vi "Test MQTT-3.1.2-1.vi"(8 "error in (no error)":errorcluster, 11 "Connection Config":refnum<class "Connection.lvclass">) -> (0 "error out":errorcluster, 3 "Connection Config dup":refnum<class "Connection.lvclass">)   [LabVIEW 2013]
uses:
  <vilib>/LabVIEW Open Source Project/MQTT Control Packets/Control Packets/CONNECT/CONNECT.lvclass
  <vilib>/LabVIEW Open Source Project/MQTT Control Packets/Control Packets/ControlPacket/ControlPacket.lvclass
  <vilib>/addons/_JKI Toolkits/Caraya/classes/Test/Test.lvclass
  <vilib>/addons/_JKI Toolkits/Caraya/classes/Assert/Assert.lvclass
  <vilib>/LabVIEW Open Source Project/Connection/Connection/Connection.lvclass
  <vilib>/LabVIEW Open Source Project/MQTT Connection/MQTT_Connection/Connection/Connection.lvclass
panel:
  out "error out 2":errorcluster
  out "connected":bool
  out "Bytes":u8[](array[numeric]) format="%08b"
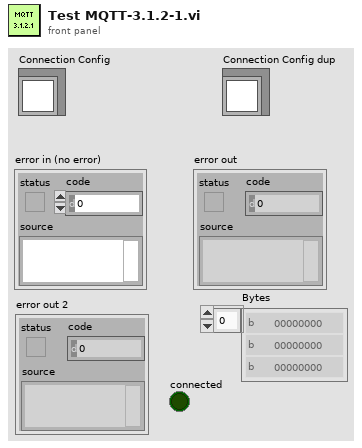
[diagram p1: front panel]
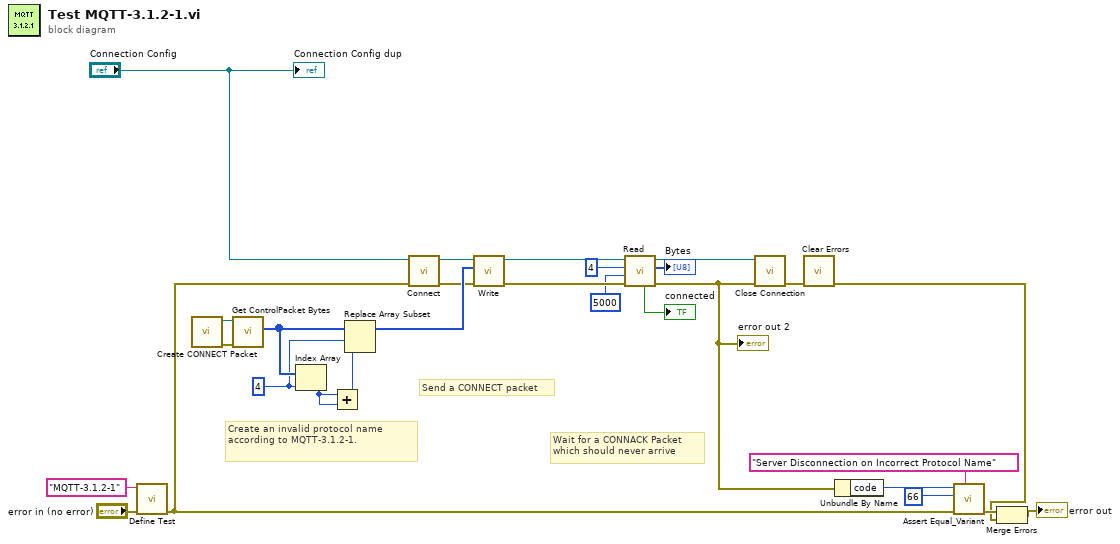
[diagram p0: block diagram]
diagram:
  w22 = 4 ("index")
  # "Wait for a CONNACK Packet\nwhich should never arrive"
  # "Create an invalid protocol name according to MQTT-3.1.2-1."
  # "Send a CONNECT packet"
  n1 = call <vilib>:"Define Test.vi"("error in (no error)"="error in (no error)", "Label (VI Title)"="MQTT-3.1.2-1") -> ("error out"=w5:errorcluster)  [unwired: 9 in]
  n2 = call <vilib>:"Create CONNECT Packet.vi"() -> ("error out"=w27:errorcluster, "CONNECT"=w28:refnum<class "CONNECT.lvclass">)  [unwired: 9 in, 1 out]
  n3 = call <vilib>:"Get ControlPacket Bytes.vi"("error in (no error)"=w27, "ControlPacket"=w28) -> ("Bytes Stream"=w24:u8[])  [unwired: 6 in, 3 out]
  n4 = Index Array(array=w24, index=w22) -> (element=w4:u8)
  n5 = Add(x=w4, y=w4) -> (x+y=w8:u8)
  n6 = Replace Array Subset(array=w24, new element=w8, index=w22) -> (w23:u8[])
  n7 = call <vilib>:"Connect.vi"("error in (no error)"=w5, "Connection in"="Connection Config") -> ("error out"=w6:errorcluster, "Connection out"=w7:refnum<class "Connection.lvclass">)  [unwired: 8 in]
  n8 = call <vilib>:"Write.vi"("error in (no error)"=w6, "Bytes"=w23, "Connection in"=w7) -> ("error out"=w25:errorcluster, "Connection"=w26:refnum<class "Connection.lvclass">)  [unwired: 7 in]
  n9 = call <vilib>:"Read.vi"("error in (no error)"=w25, "timeout (2000 ms)"=5000 ("timeout ms (25000)"), "bytes to read (100)"=4 ("bytes to read"), "TCPConnection in"=w26) -> ("error out"=w10:errorcluster, "Bytes"=→"Bytes":u8[], "TCPConnection out"=w21:refnum<class "Connection.lvclass">, "connected"=→"connected":bool)  [unwired: 3 in, 1 out]
  "error out 2" <- w10
  n10 = call <vilib>:"Close Connection.vi"("error in (no error)"=w10, "Connection in"=w21) -> ("error out"=w14:errorcluster)  [unwired: 8 in, 1 out]
  n11 = call <vilib>:"Clear Errors.vi"("error in (no error)"=w14) -> ("error out"=w9:errorcluster)  [unwired: 6 in]
  n12 = Unbundle By Name(w10) -> ("code"=w16:i32)
  n13 = call <vilib>:"Assert Equal_Variant.vi"("Label"="Server Disconnection on Incorrect Protocol Name", "error in (no error)"=w5, "Y"=66 ("code"), "X"=w16) -> ("error out"=w19:errorcluster)  [unwired: 7 in]
  n14 = Merge Errors(w19, w9) -> (→"error out":errorcluster)
  "Connection Config dup" <- "Connection Config"
